vi "Get Device Names.vi"(8 "error in (no error)":errorcluster) -> (0 "error out":errorcluster, 2 "Alias":string[](array[string]), 3 "Resource":string[](array[string]))   [LabVIEW 2025, in "I2C Bus Monitor UI.lvlib"]
uses:
  I2C Bus Monitor UI.lvlib
  <vilib>/nisyscfg/Filter Mode.ctl
  <vilib>/nisyscfg/Close (Resources).vi
  <vilib>/nisyscfg/Close (System).vi
  <resource>/objmgr/niflexrioatomicsae.rc
  <vilib>/nisyscfg/nisyscfg.lvlib
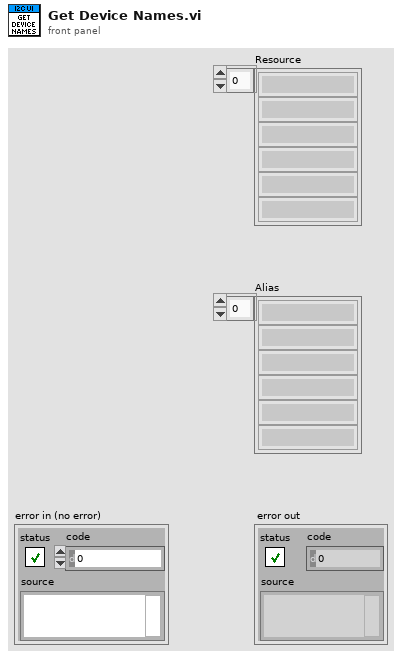
[diagram p1: front panel]
types:
  T1 = typedef "nisyscfg.lvlib/Filter Mode.ctl" = i32
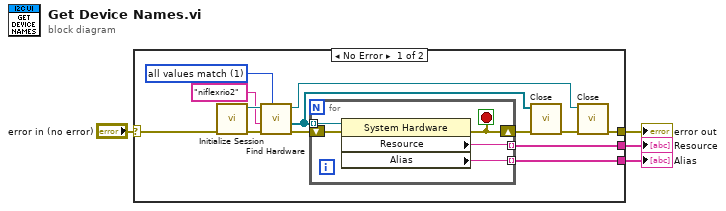
[diagram p0: block diagram]
diagram:
  n1 = case shown="No Error" "error in (no error)" {
    selector: "error in (no error)" -> [w5 w23]
    tunnel: [w9 _] -> w4
    tunnel: [w8 _] -> w3
    tunnel: [w6 w23] -> w2
    frame No Error {
      w15 = T1 1 items=["all values match"=1, "any value matches"=2, "values do not match"=3, "all properties exist"=4] ("filter mode (all values match)")
      n2 = call <vilib>:"Initialize Session.vi"("error in (no error)"=w5) -> ("error out"=w12:errorcluster, "Session out"=w16:refnum<k21>)  [unwired: 9 in]
      n3 = call <vilib>:"Find Hardware.vi"("Filter Mode (all values match)"=w15, "error in (no error)"=w12, "Experts"="niflexrio2", "Session in"=w16) -> ("error out"=w11:errorcluster, "Resources out"=w7:refnum<k20>[], "Session out"=w17:refnum<k21>)  [unwired: 1 in, 4 out]
      n4 = for {
        tunnel: w7 -> [w22] mode=indexing
        shift-right: [w18] -> w10
        shift-left: w11 -> [w19]
        tunnel: [w21] -> w9 mode=indexing
        tunnel: [w20] -> w8 mode=indexing
        stop <- w18 stop-if-true
        n5 = property class="System Hardware"(reference=w22, error in=w19) -> (error out=w18:errorcluster, "Resource"=w21:string, "Alias"=w20:string)  [unwired: 1 out]
      }
      n6 = call-poly <vilib>:"Close.vi"("error in (no error)"=w10, "Resources in"=w7) -> ("error out"=w14:errorcluster)  [unwired: 9 in]
      n7 = call-poly <vilib>:"Close.vi"("error in (no error)"=w14, "Session in"=w17) -> ("error out"=w6:errorcluster)  [unwired: 9 in]
    }
    frame Error {
    }
  }
  "Resource" <- w4
  "Alias" <- w3
  "error out" <- w2
